vi "Execute.Async.vi"(10 "parameters":variant, 11 "process":refnum<class "Process.lvclass">) -> ()   [LabVIEW 2020, in "Ballard ARINC 429 Engine.lvlib" / "Custom Device.lvlib"]
uses:
  Custom Device.lvlib
  <vilib>/NI/NIVS Inline Async API/_VS Inline Async API/Process/Process.lvclass
  Asynchronous Process Parameters.ctl
  Asynchronous Execution Unit Runtime Information.ctl
  Interfaces/Execution Unit/Execution Unit.lvclass
  Interfaces/Shared Resources/Shared Resources.lvclass
  <vilib>/NI/NIVS Inline Async API/_VS Inline Async API/Process/Process.lvclass/Process.ctl
  <vilib>/NI/NIVS Inline Async API/_Data Access Engine/Access Type Classes/ReadWrite/ReadWrite.lvclass/ReadWrite.ctl
  <vilib>/NI/NIVS Inline Async API/_Data Access Engine/Access Type Classes/Read/Read.lvclass/Read.ctl
  <vilib>/NI/NIVS Inline Async API/_Data Access Engine/Access Type Classes/Write/Write.lvclass/Write.ctl
  <vilib>/NI/NIVS Inline Async API/_VS Inline Async API/Process/Data Member Access/Read Data Access.vi
  <vilib>/NI/NIVS Inline Async API/_VS Inline Async API/Error Handling Process/SubVIs/Error.ConvertArray.vi
  <vilib>/NI/NIVS Inline Async API/_Data Access Engine/Access Type Classes/Read/Read.ProcessData.vi
  <vilib>/NI/NIVS Inline Async API/_Data Access Engine/Access Type Classes/Write/Write.ProcessData.vi
  <vilib>/NI/NIVS Inline Async API/_Data Access Engine/Access Type Classes/ReadWrite/ReadWrite.ProcessData.vi
  <vilib>/NI/NIVS Inline Async API/_Data Access Engine/Access Type Classes/Write/Write.Buffer.vi
  <vilib>/NI/NIVS Inline Async API/_Data Access Engine/Access Type Classes/Write/Write.Commit.vi
  <vilib>/NI/NIVS Inline Async API/_Data Access Engine/Data Access Engine/Data Access Engine.lvclass
  <vilib>/NI/NIVS Inline Async API/_Data Access Engine/Data Access Engine/Methods/Write.Lookup.vi
  <vilib>/NI/NIVS Inline Async API/_Data Access Engine/Data Access Engine/Methods/ReadWrite.Data.vi
  <vilib>/NI/NIVS Inline Async API/_Data Access Engine/Data Access Engine/Methods/Read.Data.vi
  <vilib>/NI/NIVS Inline Async API/_Data Access Engine/Data Access Engine/Methods/ReadWrite.Lookup.vi
  <vilib>/NI/NIVS Inline Async API/_Data Access Engine/Data Access Engine/Methods/Read.Lookup.vi
  <vilib>/NI/NIVS Inline Async API/_Data Access Engine/Data Access Engine/Methods/Write.Data.vi
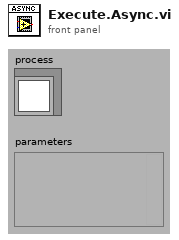
[diagram p1: front panel]
types:
  T1 = typedef "Asynchronous Process Parameters.ctl" = cluster{"Grouped Asynchronous Execution Unit Runtime Information":T2[], "shared resources":refnum<class "Shared Resources.lvclass">}
  T2 = typedef "Ballard ARINC 429 Engine.lvlib/Custom Device.lvlib/Asynchronous Execution Unit Runtime Information.ctl" = cluster{"Execution Unit":refnum<class "Execution Unit.lvclass">, "Incoming Channel Group Name":string, "Outgoing Channel Group Name":string, "ReadWrite Channel Group Name":string}
  T3 = typedef "Data Access Engine.lvlib/Data Access Engine.lvclass/Write.DVR.ctl" = refnum<data-value>
  T4 = typedef "Data Access Engine.lvlib/Data Access Engine.lvclass/ReadWrite.DVR.ctl" = refnum<data-value>
  T5 = typedef "Data Access Engine.lvlib/Data Access Engine.lvclass/Read.DVR.ctl" = refnum<data-value>
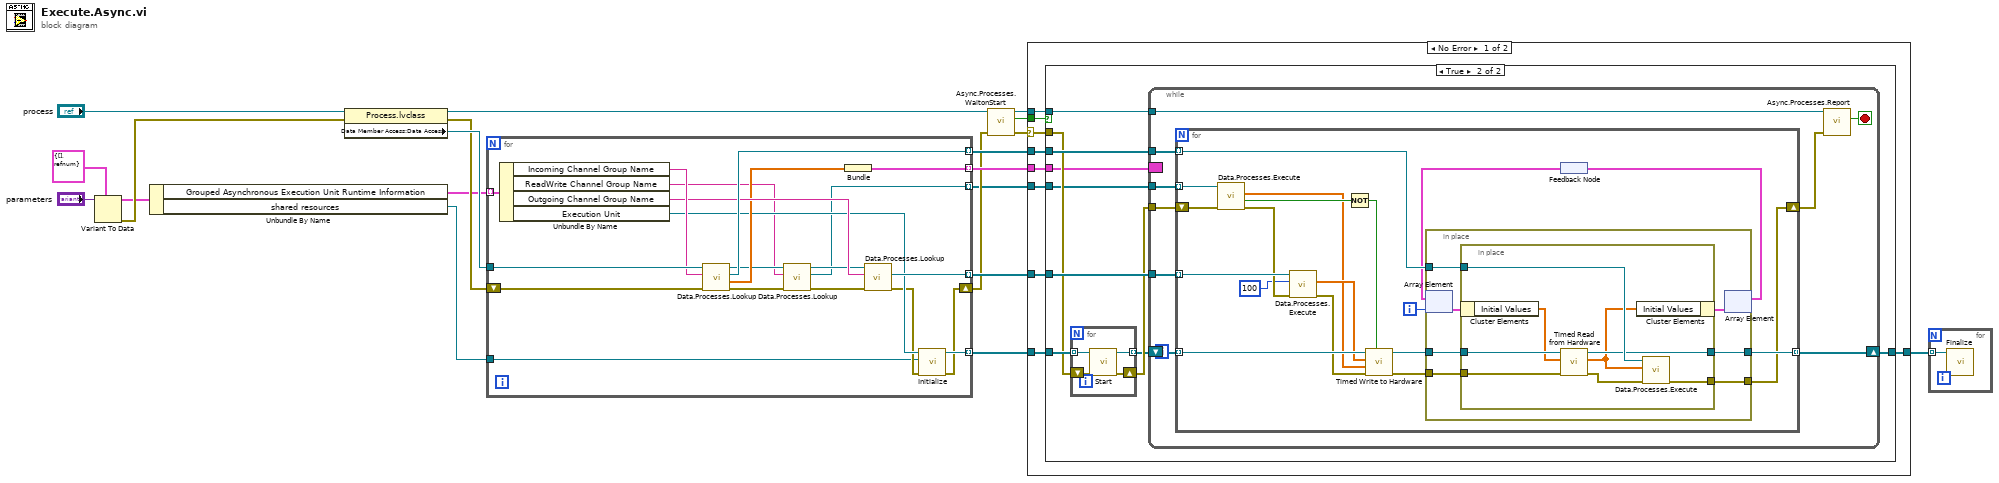
[diagram p0: block diagram]
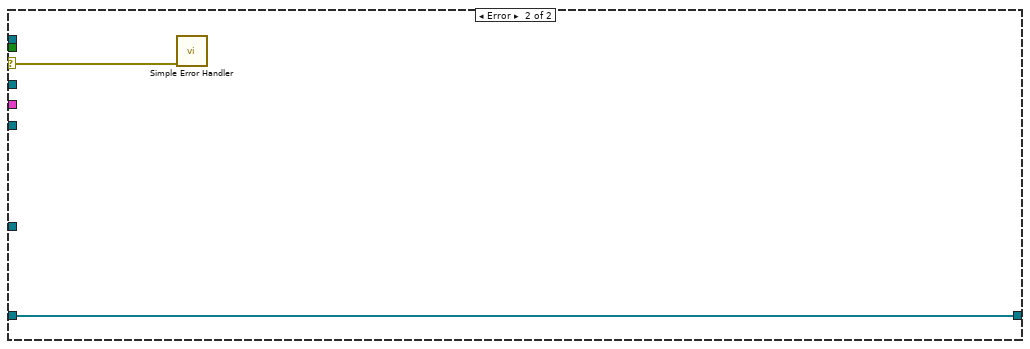
[diagram p3: hidden frame]
diagram:
  n1 = Variant To Data(type=T1 {"Grouped Asynchronous Execution Unit Runtime Information"=[], "shared resources"=refnum} ("asynchronous process parameters"), Variant="parameters") -> (data=w3:T1, error out=w10:errorcluster)  [unwired: 1 in]
  n2 = Unbundle By Name(w3) -> ("Grouped Asynchronous Execution Unit Runtime Information"=w1:T2[], "shared resources"=w2:refnum<class "Shared Resources.lvclass">)
  n3 = property class="Process.lvclass"(reference="process", error in=w10) -> (reference out=w14:refnum<class "Process.lvclass">, error out=w12:errorcluster, "Data Member Access:Data Access"=w13:refnum<class "Data Access Engine.lvclass">)
  n4 = for {
    tunnel: [w40] -> w17 mode=indexing
    tunnel: [w39] -> w16 mode=indexing
    tunnel: w13 -> [w38]
    tunnel: [w21] -> w9 mode=indexing
    tunnel: [w32] -> w8 mode=indexing
    tunnel: [w25] -> w4 mode=indexing
    shift-right: [w30] -> w7
    shift-left: w12 -> [w37]
    tunnel: w2 -> [w23]
    tunnel: w1 -> [w22] mode=indexing
    n5 = Unbundle By Name(w22) -> ("Incoming Channel Group Name"=w36:string, "ReadWrite Channel Group Name"=w24:string, "Outgoing Channel Group Name"=w35:string, "Execution Unit"=w33:refnum<class "Execution Unit.lvclass">)
    n6 = call-poly <vilib>:"Data.Processes.Lookup.vi"("error in (no error)"=w37, "Name"=w36, "Data Access API in"=w38) -> ("error out"=w29:errorcluster, "Initial Values"=w34:dbl[], "Ref"=w39:T3, "Data Access API out"=w28:refnum<class "Data Access Engine.lvclass">)  [unwired: 5 in]
    n7 = call-poly <vilib>:"Data.Processes.Lookup.vi"("error in (no error)"=w29, "Name"=w24, "Data Access API in"=w28) -> ("error out"=w26:errorcluster, "Ref"=w25:T4, "Data Access API out"=w27:refnum<class "Data Access Engine.lvclass">)  [unwired: 5 in, 1 out]
    n8 = Bundle("Initial Values"=w34) -> (w21:cluster{"Initial Values":dbl[]})  [unwired: 1 in]
    n9 = call-poly <vilib>:"Data.Processes.Lookup.vi"("error in (no error)"=w26, "Name"=w35, "Data Access API in"=w27) -> ("error out"=w31:errorcluster, "Ref"=w40:T5)  [unwired: 5 in, 2 out]
    n10 = call-dynamic "Initialize.vi"("error in"=w31, "shared resources"=w23, "Execution Unit in"=w33) -> ("error out"=w30:errorcluster, "Execution Unit out"=w32:refnum<class "Execution Unit.lvclass">)  [unwired: 7 in]
  }
  n11 = call <vilib>:"Async.Processes.WaitonStart.vi"("error in (no error)"=w7, "Process"=w14) -> ("error out"=w18:errorcluster, "Execute"=w20:bool, "Process out"=w19:refnum<class "Process.lvclass">)  [unwired: 7 in]
  n12 = case shown="No Error" w18 {
    selector: w18 -> [w45 w109]
    tunnel: w20 -> [w49 _]
    tunnel: w19 -> [w48 _]
    tunnel: w16 -> [w47 _]
    tunnel: w17 -> [w46 _]
    tunnel: w9 -> [w44 _]
    tunnel: w8 -> [w43 w108]
    tunnel: [w42 w108] -> w6
    tunnel: w4 -> [w41 _]
    frame No Error {
      n13 = case shown="True" w49 {
        tunnel: w45 -> [_ w56]
        tunnel: w48 -> [_ w58]
        tunnel: w46 -> [_ w60]
        tunnel: w47 -> [_ w59]
        tunnel: w44 -> [_ w53]
        tunnel: w43 -> [w50 w57]
        tunnel: [w50 w52] -> w42
        tunnel: w41 -> [_ w51]
        frame False {
        }
        frame True {
          n14 = for {
            tunnel: w57 -> [w64] mode=indexing
            tunnel: [w61] -> w54 mode=indexing
            shift-right: [w62] -> w55
            shift-left: w56 -> [w63]
            n15 = call-dynamic "Start.vi"("error in (no error)"=w63, "Execution Unit in"=w64) -> ("error out"=w62:errorcluster, "Execution Unit out"=w61:refnum<class "Execution Unit.lvclass">)  [unwired: 8 in]
          }
          n16 = while {
            tunnel: w55 -> [w65]
            tunnel: w58 -> [w73]
            tunnel: w60 -> [w71]
            tunnel: w59 -> [w70]
            border: w53 -> [_]
            shift-right: [w68] -> w52
            shift-left: w54 -> [w69]
            tunnel: w51 -> [w67]
            stop <- w72 stop-if-true
            n17 = for {
              tunnel: w71 -> [w92] mode=indexing
              tunnel: w70 -> [w91] mode=indexing
              tunnel: w69 -> [w90] mode=indexing
              tunnel: [w87] -> w68 mode=indexing
              tunnel: w67 -> [w86] mode=indexing
              shift-right: [w85] -> w66
              shift-left: w65 -> [w77]
              i -> [w76]
              n18 = call-poly <vilib>:"Data.Processes.Execute.vi"("error in (no error)"=w77, "Ref"=w86) -> ("error out"=w84:errorcluster, "Timeout?"=w82:bool, "Data"=w78:dbl[])  [unwired: 6 in, 1 out]
              n19 = call-poly <vilib>:"Data.Processes.Execute.vi"("error in (no error)"=w84, "timeout ms"=100, "Ref"=w92) -> ("error out"=w88:errorcluster, "Values"=w79:dbl[])  [unwired: 6 in, 1 out]
              n20 = Not(x=w82) -> (.not. x?=w80:bool)
              n21 = call "Timed Write to Hardware.vi"("Triggers Valid"=w80, "error in"=w88, "Trigger Values"=w78, "Values"=w79, "Execution Unit in"=w90) -> ("error out"=w83:errorcluster, "Execution Unit out"=w89:refnum<class "Execution Unit.lvclass">)  [unwired: 3 in, 2 out]
              n22 = feedback #1() -> (w75:cluster{"Initial Values":dbl[]}[])
              n23 = in-place {
                in-place-border: w91 -> [w99]
                in-place-border: w89 -> [w98]
                in-place-border: [w97] -> w87
                in-place-border: [w96] -> w85
                in-place-border: w83 -> [w95]
                n24 = in-place-array #2(w75, w76) -> (w94:cluster{"Initial Values":dbl[]})
                n25 = in-place {
                  in-place-border: w99 -> [w107]
                  in-place-border: w98 -> [w106]
                  in-place-border: [w104] -> w97
                  in-place-border: [w103] -> w96
                  in-place-border: w95 -> [w102]
                  n26 = in-place-cluster #3(w94) -> ("Initial Values"=w101:dbl[])
                  n27 = call "Timed Read from Hardware.vi"("error in"=w102, "Values in"=w101, "Execution Unit in"=w106) -> ("error out"=w105:errorcluster, "Values out"=w100:dbl[], "Execution Unit out"=w104:refnum<class "Execution Unit.lvclass">)  [unwired: 6 in]
                  n28 = in-place-cluster #3("Initial Values"=w100) -> (w93:cluster{"Initial Values":dbl[]})
                  n29 = call-poly <vilib>:"Data.Processes.Execute.vi"("error in (no error)"=w105, "Values"=w100, "Ref"=w107) -> ("error out"=w103:errorcluster)  [unwired: 8 in]
                }
                n30 = in-place-array #2(w93) -> (w74:cluster{"Initial Values":dbl[]}[])  [unwired: 1 out]
              }
              n31 = feedback-in #1(w74) -> ()
            }
            n32 = call <vilib>:"Async.Processes.Report.vi"("Error"=w66, "Process in"=w73) -> ("Stop"=w72:bool)  [unwired: 8 in, 1 out]
          }
        }
      }
    }
    frame Error {
      n33 = call <vilib>:"Simple Error Handler.vi"("error in (no error)"=w109) -> ()  [unwired: 4 in, 5 out]
    }
  }
  n34 = for {
    tunnel: w6 -> [w110] mode=indexing
    n35 = call-dynamic "Finalize.vi"("Execution Unit in"=w110) -> ()  [unwired: 9 in, 2 out]
  }
